vi "Connect to Server.vi"(4 "timeout (2000 ms)":i32=2000, 5 "Connect Flags":T3={"Reserved"=FALSE, "Clean Session"=TRUE, "Will Flag"=FALSE, "Will QoS 1"=FALSE, "Will QoS 2"=FALSE, "Will Retain"=FALSE, "Password Flag"=FALSE, "User Name Flag"=FALSE}, 6 "Keep Alive (s)":u16=60, 7 "Payload":T2, 8 "error in (no error)":errorcluster, 11 "Client in":refnum<class "Client.lvclass">) -> (0 "error out":errorcluster, 1 "timed out":bool, 2 "Return Code":T1=enum."Server Unavailable", 3 "Client out":refnum<class "Client.lvclass">)   [LabVIEW 2013, in "MQTT Client.lvlib" / "Client.lvclass"]
uses:
  Client.lvclass
  <vilib>/LabVIEW Open Source Project/MQTT Control Packets/Control Packets/CONNECT/ConnectFlags -- cluster.ctl
  <vilib>/LabVIEW Open Source Project/MQTT Control Packets/Control Packets/CONNACK/Connect Return Code -- enum.ctl
  <vilib>/LabVIEW Open Source Project/MQTT Control Packets/Control Packets/CONNACK/CONNACK.lvclass
  <vilib>/LabVIEW Open Source Project/MQTT Connection/MQTT_Base/Base Class/MQTT_Base.lvclass/MQTT_Base.ctl
  Client.lvclass/Client.ctl
  <vilib>/LabVIEW Open Source Project/MQTT Control Packets/Control Packets/ControlPacket/ControlPacket.lvclass
  <vilib>/LabVIEW Open Source Project/MQTT Control Packets/Control Packets/CONNECT/CONNECT.lvclass
  <vilib>/LabVIEW Open Source Project/MQTT Connection/MQTT_Base/Session/Session.lvclass
  <vilib>/LabVIEW Open Source Project/MQTT Connection/MQTT_Base/Base Class/MQTT_Base.lvclass
  Session.Client/Session.Client.lvclass
  <vilib>/LabVIEW Open Source Project/Connection/Connection/Connection.lvclass
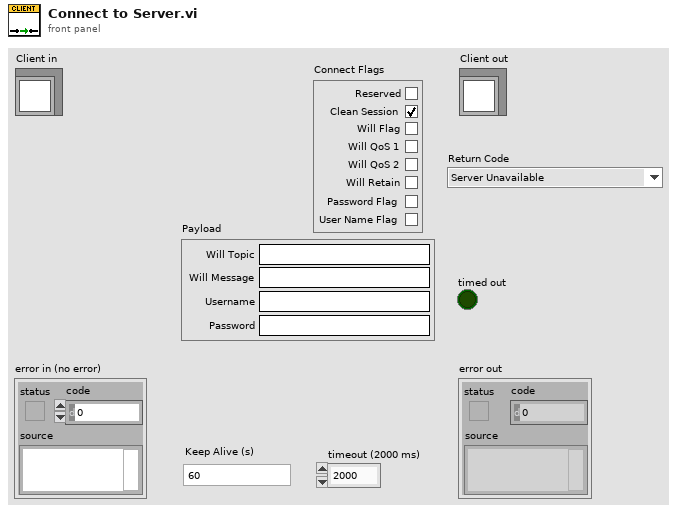
[diagram p1: front panel]
types:
  T1 = typedef "MQTT_Control_Packets.lvlib/CONNACK.lvclass/Connect Return Code -- enum.ctl" = enum16{"Connection accepted", "Unacceptable protocol version", "Identifier Rejected", "Server Unavailable", "Bad Username or Password", "Not Authorized"}
  T2 = cluster{"Will Topic":string, "Will Message":string, "Username":string, "Password":string}
  T3 = typedef "MQTT_Control_Packets.lvlib/CONNECT.lvclass/ConnectFlags -- cluster.ctl" = cluster{"Reserved":bool, "Clean Session":bool, "Will Flag":bool, "Will QoS 1":bool, "Will QoS 2":bool, "Will Retain":bool, "Password Flag":bool, "User Name Flag":bool}
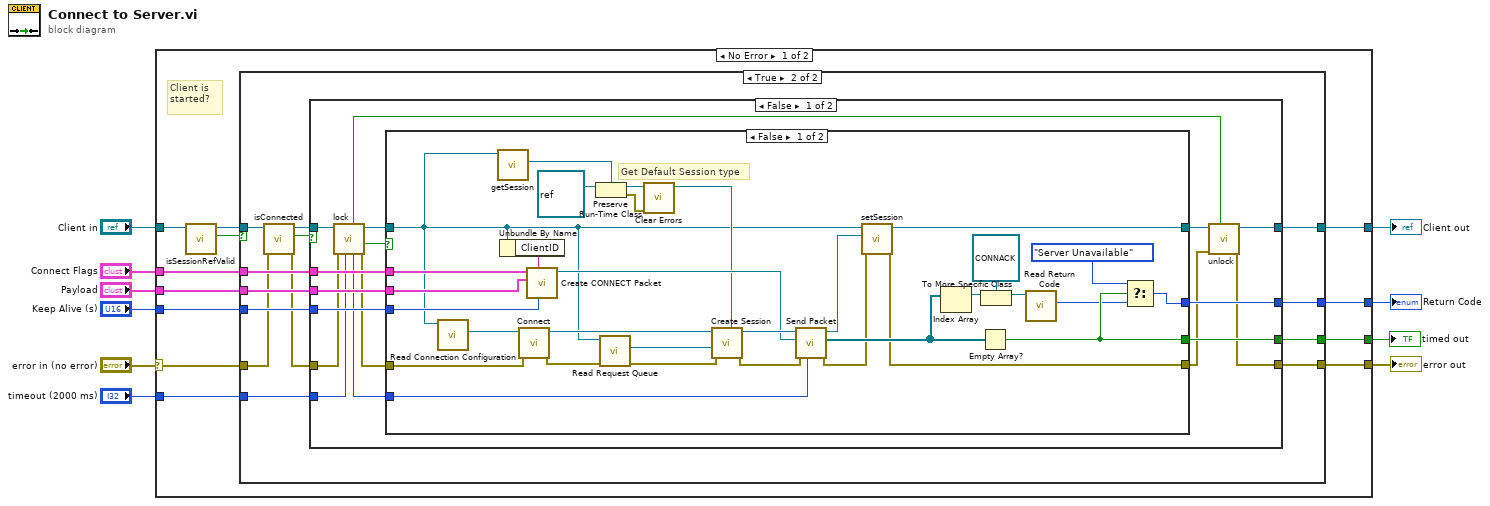
[diagram p0: block diagram]
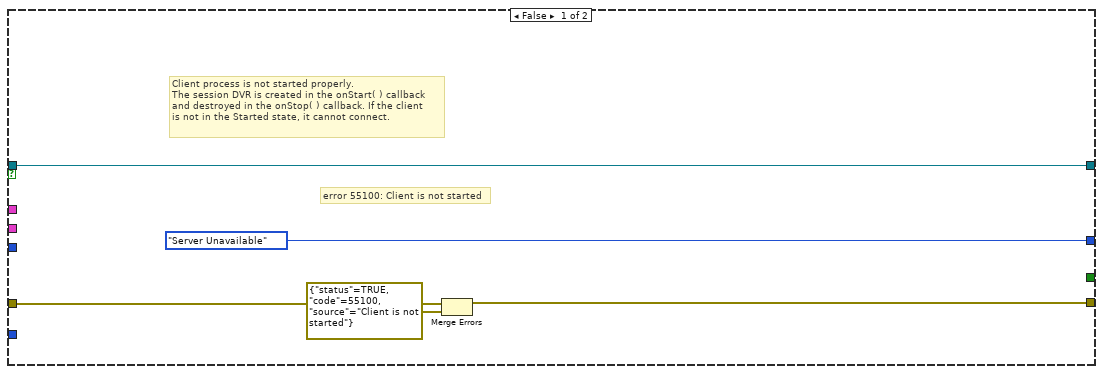
[diagram p2: hidden frame]
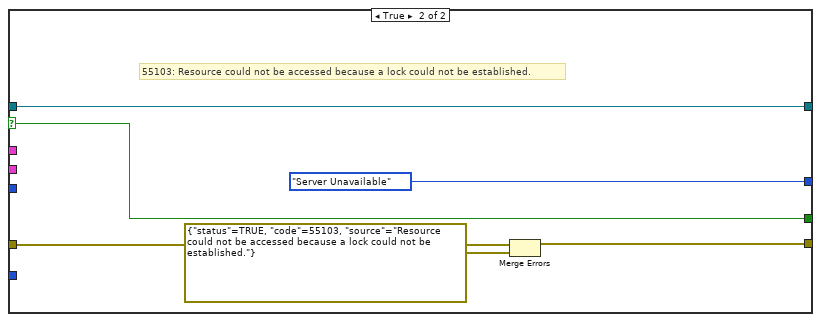
[diagram p3: hidden frame]
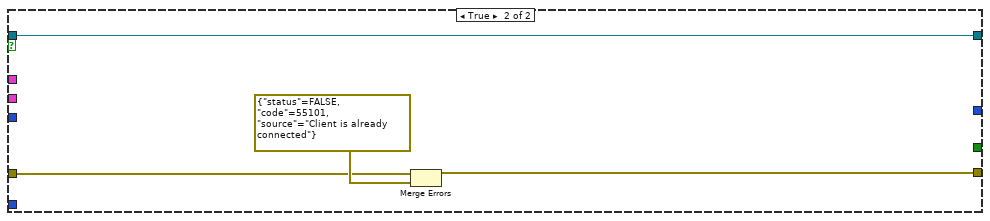
[diagram p4: hidden frame]
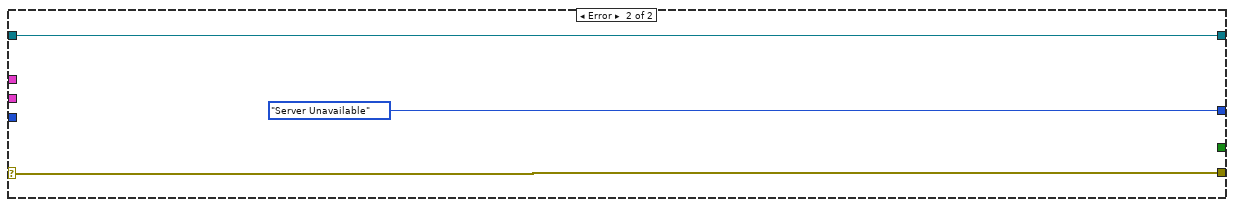
[diagram p5: hidden frame]
diagram:
  n1 = case shown="No Error" "error in (no error)" {
    selector: "error in (no error)" -> [w14 w101]
    tunnel: [w15 w101] -> w9
    tunnel: [w22 w100] -> w7
    tunnel: "Client in" -> [w13 w100]
    tunnel: "Connect Flags" -> [w21 _]
    tunnel: "Payload" -> [w20 _]
    tunnel: "Keep Alive (s)" -> [w19 _]
    tunnel: [w16 _] -> w3
    tunnel: "timeout (2000 ms)" -> [w18 _]
    tunnel: [w17 Connect_Return_Code_--_enum."Server Unavailable" ("Return Code")] -> w1
    frame No Error {
      # "Client is started?"
      n2 = call "isSessionRefValid.vi"("Client in"=w13) -> ("Session ref valid"=w11:bool, "Client out"=w12:refnum<class "Client.lvclass">)  [unwired: 9 in]
      n3 = case shown="True" w11 {
        tunnel: [w24 w30] -> w22
        tunnel: w21 -> [_ w40]
        tunnel: w20 -> [_ w39]
        tunnel: w19 -> [_ w38]
        tunnel: w18 -> [_ w37]
        tunnel: [Connect_Return_Code_--_enum."Server Unavailable" ("Return Code") w36] -> w17
        tunnel: [_ w35] -> w16
        tunnel: [w26 w29] -> w15
        tunnel: w14 -> [w27 w33]
        tunnel: w12 -> [w24 w34]
        frame False {
          # "error 55100: Client is not started"
          # "Client process is not started properly.\nThe session DVR is created in the onStart( ) callback\nand destroyed in the onStop( ) callback. If the client\nis not in the Started state, it cannot connect."
          n4 = Merge Errors(w27, errorcluster {"status"=TRUE, "code"=55100, "source"="Client is not started"} ("error in")) -> (w26:errorcluster)
        }
        frame True {
          n5 = call "isConnected.vi"("error in (no error)"=w33, "Client in"=w34) -> ("error out"=w32:errorcluster, "connected"=w28:bool, "Client out"=w31:refnum<class "Client.lvclass">)  [unwired: 7 in]
          n6 = case shown="False" w28 {
            tunnel: w40 -> [w57 _]
            tunnel: w39 -> [w56 _]
            tunnel: w38 -> [w55 _]
            tunnel: w37 -> [w50 _]
            tunnel: [w54 _] -> w36
            tunnel: [w53 _] -> w35
            tunnel: w32 -> [w48 w97]
            tunnel: w31 -> [w52 w95]
            tunnel: [w45 w95] -> w30
            tunnel: [w43 w96] -> w29
            frame False {
              n7 = call "lock.vi"("timeout (2000ms)"=w50, "error in (no error)"=w48, "Client in"=w52) -> ("error out"=w47:errorcluster, "timed out"=w41:bool, "Client out"=w51:refnum<class "Client.lvclass">, "remaining (ms)"=w49:i32, "locked"=w42:bool)  [unwired: 4 in]
              n8 = case shown="False" w41 {
                selector: w41 -> [_ w92]
                tunnel: w57 -> [w88 _]
                tunnel: w56 -> [w87 _]
                tunnel: w55 -> [w86 _]
                tunnel: [w58 Connect_Return_Code_--_enum."Server Unavailable" ("Return Code")] -> w54
                tunnel: [w61 w92] -> w53
                tunnel: w51 -> [w66 w94]
                tunnel: w49 -> [w65 _]
                tunnel: w47 -> [w64 w91]
                tunnel: [w63 w94] -> w46
                tunnel: [w62 w90] -> w44
                frame False {
                  # "Get Default Session type"
                  n9 = call <vilib>:"Read Connection Configuration.vi"("MQTT_Base in"=w66) -> ("Connection Configuration"=w73:refnum<class "Connection.lvclass">)  [unwired: 8 in, 2 out]
                  n10 = call "getSession.vi"("Client in"=w66) -> ("Session"=w69:refnum<class "Session.Client.lvclass">)  [unwired: 8 in, 2 out]
                  n11 = Unbundle By Name(w66) -> ("ClientID"=w85:string)
                  n12 = call <vilib>:"Connect.vi"("error in (no error)"=w64, "Connection in"=w73) -> ("error out"=w75:errorcluster, "Connection out"=w74:refnum<class "Connection.lvclass">)  [unwired: 8 in]
                  n13 = call <vilib>:"Create CONNECT Packet.vi"("Keep Alive (s)"=w86, "Client ID (empty: generate new)"=w85, "Payload"=w87, "Connect Flags"=w88) -> ("CONNECT"=w82:refnum<class "CONNECT.lvclass">)  [unwired: 5 in, 2 out]
                  n14 = Preserve Run-Time Class(object in=refnum<class> refnum ("LabVIEW Object"), 2:w69) -> (object out=w67:refnum<class "Session.Client.lvclass">, error out=w68:errorcluster)  [unwired: 1 in]
                  n15 = call <vilib>:"Read Request Queue.vi"("error in (no error)"=w75, "MQTT_Base in"=w66) -> ("error out"=w77:errorcluster, "Request"=w84:refnum<queue>)  [unwired: 7 in, 1 out]
                  n16 = call <vilib>:"Clear Errors.vi"("error in (no error)"=w68) -> ()  [unwired: 6 in, 1 out]
                  n17 = call <vilib>:"Create Session.vi"("Session in"=w67, "error in (no error)"=w77, "Request"=w84, "Connection"=w74) -> ("error out"=w76:errorcluster, "Session"=w83:refnum<class "Session.Client.lvclass">)  [unwired: 6 in]
                  n18 = call "Send Packet.vi"("timeout (0ms : no ack)"=w65, "error in (no error)"=w76, "Packet"=w82, "Session"=w83) -> ("error out"=w71:errorcluster, "Response"=w78:refnum<class "ControlPacket.lvclass">[], "Session"=w72:refnum<class "Session.Client.lvclass">)  [unwired: 4 in, 1 out]
                  n19 = call "setSession.vi"("error in (no error)"=w71, "Session"=w72, "Client in"=w66) -> ("error out"=w62:errorcluster, "Client out"=w63:refnum<class "Client.lvclass">)  [unwired: 7 in]
                  n20 = Index Array(array=w78) -> (element=w81:refnum<class "ControlPacket.lvclass">)  [unwired: 1 in]
                  n21 = Empty Array?(array=w78) -> (empty?=w61:bool)
                  n22 = To More Specific Class(target class=refnum<class "CONNACK.lvclass"> refnum ("CONNACK.lvclass"), reference=w81) -> (specific class reference=w79:refnum<class "CONNACK.lvclass">)  [unwired: 1 in, 1 out]
                  n23 = call <vilib>:"Read Return Code.vi"("CONNACK in"=w79) -> ("Return Code"=w59:T1)  [unwired: 8 in, 2 out]
                  n24 = Select(t=Connect_Return_Code_--_enum."Server Unavailable" ("Return Code"), s=w61, f=w59) -> (s? t:f=w58:T1)
                }
                frame True {
                  # "55103: Resource could not be accessed because a lock could not be established."
                  n25 = Merge Errors(w91, errorcluster {"status"=TRUE, "code"=55103, "source"="Resource could not be accessed because a lock could not be established."} ("error in")) -> (w90:errorcluster)
                }
              }
              n26 = call "unlock.vi"("Unlock?"=w42, "error in (no error)"=w44, "Client in"=w46) -> ("error out"=w43:errorcluster, "Client out"=w45:refnum<class "Client.lvclass">)  [unwired: 7 in]
            }
            frame True {
              n27 = Merge Errors(w97, errorcluster {"status"=FALSE, "code"=55101, "source"="Client is already connected"} ("error in")) -> (w96:errorcluster)
            }
          }
        }
      }
    }
    frame Error {
    }
  }
  "error out" <- w9
  "Client out" <- w7
  "timed out" <- w3
  "Return Code" <- w1
